vi "Open GUI.vi"(8 "error in (no error)":errorcluster, 11 "PluginGUI in":refnum<class "PluginGUI.lvclass">) -> (0 "error out":errorcluster, 3 "PluginGUI out":refnum<class "PluginGUI.lvclass">)   [LabVIEW 2020, in "VolatusGUI.lvlib" / "PluginGUI.lvclass"]
uses:
  PluginGUI.lvclass
  Visibility Data.ctl
  PluginGUI.lvclass/PluginGUI.ctl
  Volatus/MessageQ/MessageQ.lvclass/MessageQ.ctl
  VolatusGUI.lvlib
  Volatus/MessageQ/MessageQ.lvclass
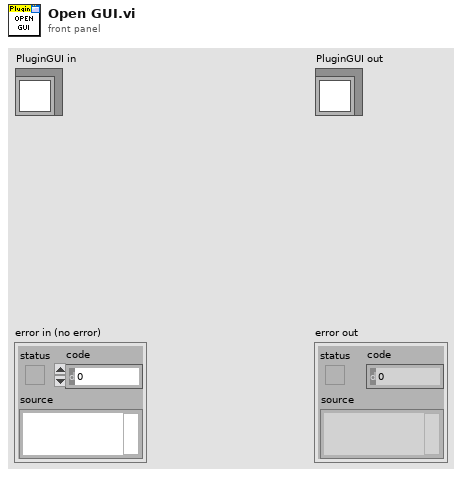
[diagram p1: front panel]
types:
  T1 = typedef "VolatusGUI.lvlib/Visibility Data.ctl" = cluster{"GUI ID":string, "Visible":bool}
  T2 = enum32{"Invalid", "Standard", "Closed", "Hidden", "Minimized", "Maximized"}
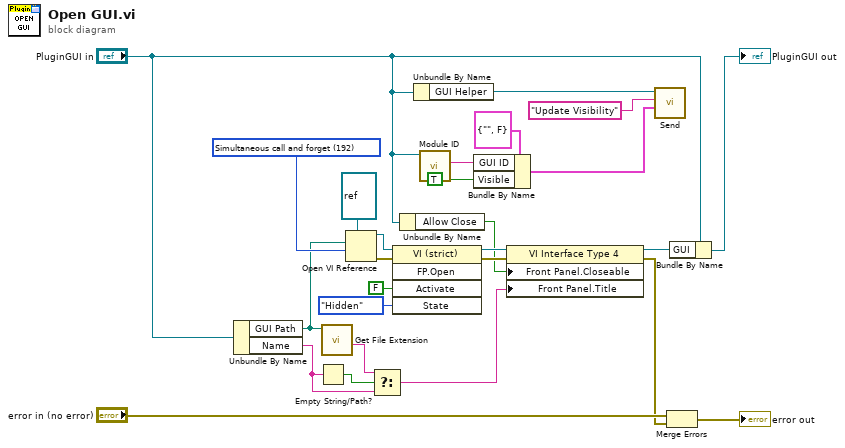
[diagram p0: block diagram]
diagram:
  w25 = 192 items=["Record modifications"=1, "Open templates for editing"=2, "Prompt user to save"=4, "Prepare for reentrant run"=8, "Prompt to find missing subVIs"=16, "Hide loading dialog box"=32, "Enable simultaneous calls"=64, "Prepare to call and forget"=128, "Simultaneous call and forget"=192, "Prepare to call and collect"=256, "Simultaneous call and collect"=320]
  n1 = Unbundle By Name("PluginGUI in") -> ("GUI Path"=w5:path, "Name"=w3:string)
  n2 = Empty String/Path?(string/path=w3) -> (empty?=w4:bool)
  n3 = call <vilib>:"Get File Extension.vi"("file"=w5) -> ("filename without extension"=w2:string)  [unwired: 6 in, 4 out]
  n4 = Open VI Reference(type specifier VI Refnum (for type only)=refnum<vi> refnum, vi path=w5, options=w25) -> (vi reference=w20:refnum<vi>, error out=w21:errorcluster)  [unwired: 3 in]
  n5 = Select(t=w2, s=w4, f=w3) -> (s? t:f=w1:string)
  n6 = invoke class="VI (strict)" method="FP.Open"(reference=w20, error in=w21, "Activate"=FALSE ("Activate?"), "State"=T2."Hidden") -> (reference out=w17:refnum<vi>, error out=w16:errorcluster)  [unwired: 1 in, 3 out]
  n7 = Unbundle By Name("PluginGUI in") -> ("Allow Close"=w15:bool)
  n8 = Unbundle By Name("PluginGUI in") -> ("GUI Helper"=w9:refnum<class "MessageQ.lvclass">)
  n9 = call-dynamic "Module ID.vi"("PluginGUI in"="PluginGUI in") -> ("Module ID"=w10:string)  [unwired: 10 in]
  n10 = Bundle By Name(cluster=T1 {"GUI ID"="", "Visible"=FALSE} ("Visibility Data"), "GUI ID"=w10, "Visible"=TRUE) -> (w8:T1)
  n11 = property class="VI Interface Type 4"(reference=w17, error in=w16, "Front Panel.Closeable"=w15, "Front Panel.Title"=w1) -> (reference out=w14:refnum<vi>, error out=w13:errorcluster)
  n12 = call "Send.vi"("Data"=w8, "ID"="Update Visibility", "MessageQ in"=w9) -> ()  [unwired: 7 in, 2 out]
  n13 = Merge Errors("error in (no error)", w13) -> (→"error out":errorcluster)
  n14 = Bundle By Name(cluster="PluginGUI in", "GUI"=w14) -> (→"PluginGUI out":refnum<class "PluginGUI.lvclass">)
